vi "Echo_Send_Echo.vi"(4 "n frames":i32, 5 "buffers":T5, 6 "frame":T3 {"id" format="%.0x"}, 7 "context":T6 {"ack hi" format="%.0x"; "ack lo" format="%.0x"; "test hi" format="%.0x"; "test lo" format="%.0x"}, 8 "error in (no error)":errorcluster, 9 "counters in":T1, 10 "time store in":T2, 11 "tx in":u8[](array[numeric])) -> (0 "error out":errorcluster, 1 "counters out":T1, 2 "time store out":T2, 3 "tx out":u8[](array[numeric]))   [LabVIEW 2021]
doc: "S5 echo, Test case: sends the echo of frame index with W14 at ID + echo offset (keeps IDE/FDF/BRS), time-stamps around the TCP Write (High Resolution Relative Seconds), stores t_dev, t_rx_lv, t_send_lv at key, increments echoes sent. tx and time store change in place."
uses:
  CANsub_C.lvlib
  Echo_Time_Store.ctl
  Echo_Counters.ctl
  Echo_Context.ctl
  C_RX_Buffers.ctl
  Echo_Frame_Kind.ctl
  Echo_Frame.ctl
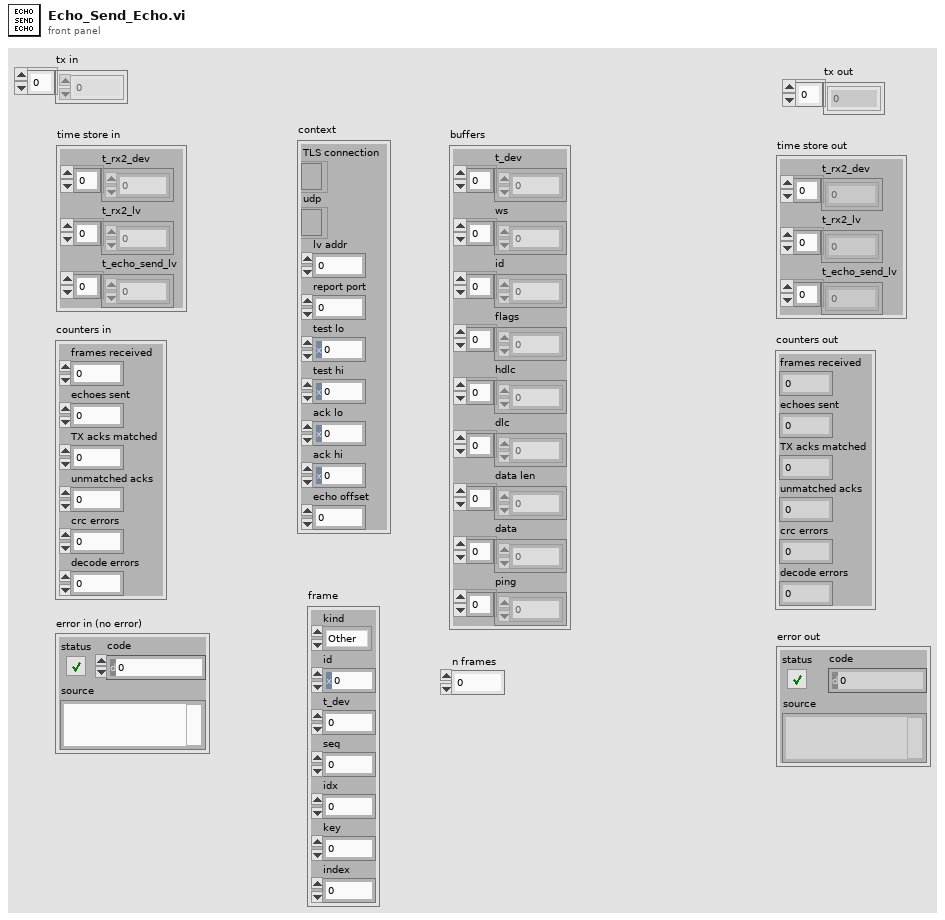
[diagram p1: front panel]
types:
  T1 = typedef "Echo_Counters.ctl" = cluster{"frames received":u32, "echoes sent":u32, "TX acks matched":u32, "unmatched acks":u32, "crc errors":u32, "decode errors":i32}
  T2 = typedef "Echo_Time_Store.ctl" = cluster{"t_rx2_dev":dbl[], "t_rx2_lv":dbl[], "t_echo_send_lv":dbl[]}
  T3 = typedef "Echo_Frame.ctl" = cluster{"kind":T4, "id":u32, "t_dev":dbl, "seq":u16, "idx":u8, "key":i32, "index":i32}
  T4 = typedef "Echo_Frame_Kind.ctl" = enum16{"Other", "Test", "Ack"}
  T5 = typedef "CANsub_C.lvlib/C_RX_Buffers.ctl" = cluster{"t_dev":dbl[], "ws":u8[], "id":u32[], "flags":u16[], "hdlc":u8[], "dlc":u8[], "data len":u8[], "data":u8[], "ping":u8[]}
  T6 = typedef "Echo_Context.ctl" = cluster{"TLS connection":refnum<k5>, "udp":refnum<k16>, "lv addr":u32, "report port":u16, "test lo":u32, "test hi":u32, "ack lo":u32, "ack hi":u32, "echo offset":i32}
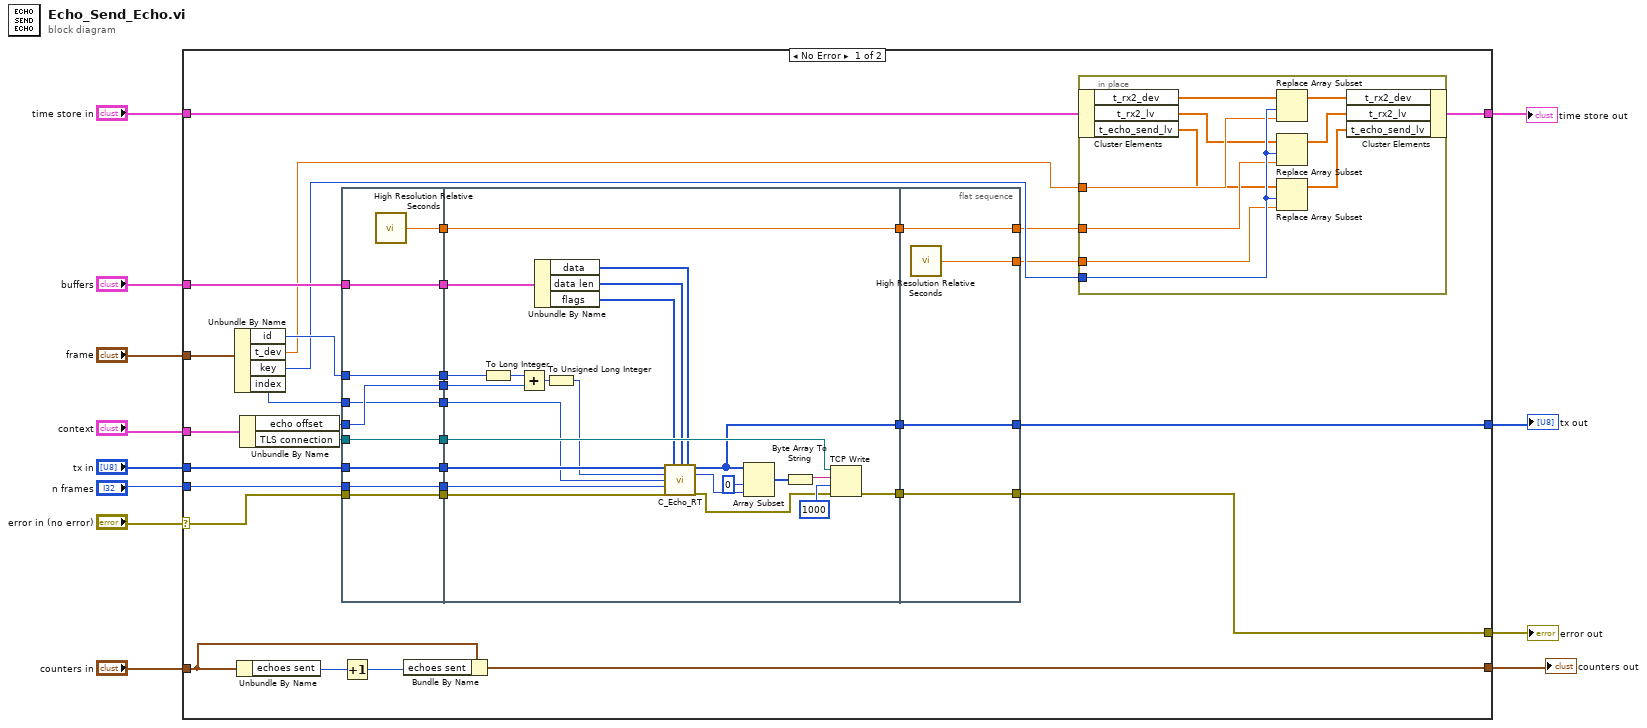
[diagram p0: block diagram]
diagram:
  n1 = case shown="No Error" "error in (no error)" {
    selector: "error in (no error)" -> [w27 w96]
    tunnel: [w13 w96] -> w11
    tunnel: [w18 w95] -> w10
    tunnel: "tx in" -> [w36 w95]
    tunnel: [w19 w94] -> w8
    tunnel: "time store in" -> [w24 w94]
    tunnel: [w14 w93] -> w6
    tunnel: "counters in" -> [w16 w93]
    tunnel: "frame" -> [w45 _]
    tunnel: "context" -> [w44 _]
    tunnel: "n frames" -> [w34 _]
    tunnel: "buffers" -> [w29 _]
    frame No Error {
      n2 = Unbundle By Name(w45) -> ("id"=w42:u32, "t_dev"=w23:dbl, "key"=w22:i32, "index"=w32:i32)
      n3 = Unbundle By Name(w16) -> ("echoes sent"=w17:u32)
      n4 = Unbundle By Name(w44) -> ("echo offset"=w39:i32, "TLS connection"=w37:refnum<k5>)
      n5 = flat-sequence {
        tunnel: [w65] -> w46
        tunnel: w42 -> [w64]
        tunnel: [w64] -> w41
        tunnel: [w63] -> w40
        tunnel: w39 -> [w63]
        tunnel: [w62] -> w38
        tunnel: w37 -> [w62]
        tunnel: w36 -> [w61]
        tunnel: [w61] -> w35
        tunnel: w34 -> [w60]
        tunnel: [w60] -> w33
        tunnel: w32 -> [w59]
        tunnel: [w59] -> w31
        tunnel: [w58] -> w30
        tunnel: w29 -> [w58]
        tunnel: [w57] -> w28
        tunnel: w27 -> [w57]
        tunnel: w46 -> [w88]
        tunnel: [w88] -> w43
        tunnel: w41 -> [w82]
        tunnel: w40 -> [w80]
        tunnel: w38 -> [w79]
        tunnel: w35 -> [w78]
        tunnel: w33 -> [w75]
        tunnel: w31 -> [w74]
        tunnel: w30 -> [w73]
        tunnel: w28 -> [w69]
        tunnel: [w67] -> w26
        tunnel: [w66] -> w25
        tunnel: [w92] -> w20
        tunnel: w43 -> [w92]
        tunnel: [w91] -> w21
        tunnel: [w90] -> w13
        tunnel: w26 -> [w90]
        tunnel: [w89] -> w18
        tunnel: w25 -> [w89]
        frame #0 {
          n6 = call <vilib>:"High Resolution Relative Seconds.vi"() -> ("relative seconds"=w65:dbl)
        }
        frame #1 {
          n7 = To Long Integer(number=w82) -> (32bit integer=w81:i32)
          n8 = Add(x=w81, y=w80) -> (x+y=w77:i32)
          n9 = Unbundle By Name(w73) -> ("data"=w70:u8[], "data len"=w71:u8[], "flags"=w72:u16[])
          n10 = To Unsigned Long Integer(number=w77) -> (unsigned 32bit integer=w76:u32)
          n11 = call "C_Echo_RT.vi"("tx in"=w78, "flags"=w72, "data len"=w71, "data"=w70, "new id"=w76, "index"=w74, "n frames"=w75, "error in (no error)"=w69) -> ("tx out"=w66:u8[], "length"=w87:i32, "error out"=w68:errorcluster)  [unwired: 5 in]
          n12 = Array Subset(array=w66, index=0, length=w87) -> (w85:u8[])
          n13 = Byte Array To String(unsigned byte array=w85) -> (string=w84:string)
          n14 = TCP Write(connection ID=w79, data in=w84, error in (no error)=w68, 9:1000 ("timeout ms (25000)")) -> (error out=w67:errorcluster)  [unwired: 2 out]
        }
        frame #2 {
          n15 = call <vilib>:"High Resolution Relative Seconds.vi"() -> ("relative seconds"=w91:dbl)
        }
      }
      n16 = Increment(x=w17) -> (x+1=w15:u32)
      n17 = Bundle By Name(cluster=w16, "echoes sent"=w15) -> (w14:T1)
      n18 = in-place {
        in-place-border: w23 -> [w54]
        in-place-border: w22 -> [w56]
        in-place-border: w21 -> [w55]
        in-place-border: w20 -> [w53]
        n19 = in-place-cluster #1(w24) -> ("t_rx2_dev"=w52:dbl[], "t_rx2_lv"=w51:dbl[], "t_echo_send_lv"=w50:dbl[])
        n20 = Replace Array Subset(array=w52, new element=w54, index=w56) -> (w49:dbl[])
        n21 = Replace Array Subset(array=w51, new element=w53, index=w56) -> (w48:dbl[])
        n22 = Replace Array Subset(array=w50, new element=w55, index=w56) -> (w47:dbl[])
        n23 = in-place-cluster #1("t_rx2_dev"=w49, "t_rx2_lv"=w48, "t_echo_send_lv"=w47) -> (w19:T2)
      }
    }
    frame Error {
    }
  }
  "tx out" <- w10
  "time store out" <- w8
  "counters out" <- w6
  "error out" <- w11
